vi "translation_control_panel.vi"() -> ()   [LabVIEW 2026]
panel:
  in  "?":bool
  in  "Run":bool
  out "Output":string
  in  "Output File Name":string
  in  "Timeline File":path
  in  "Translation Working Directory":path
  in  "Topology File":path
  in  ".mat File Directory":path
  out "Command Preview":string
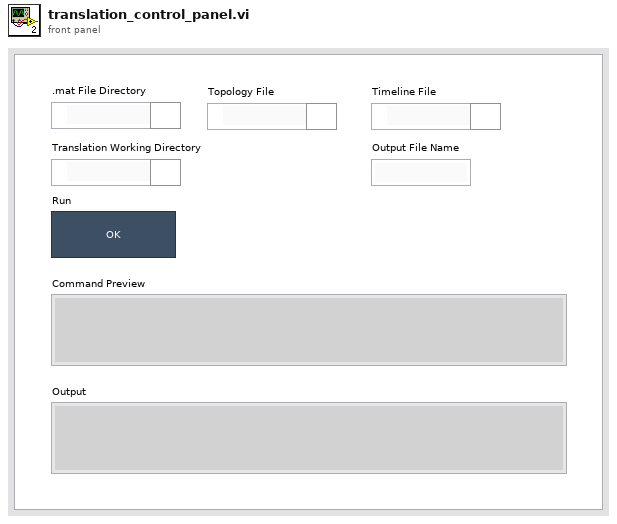
[diagram p1: front panel]
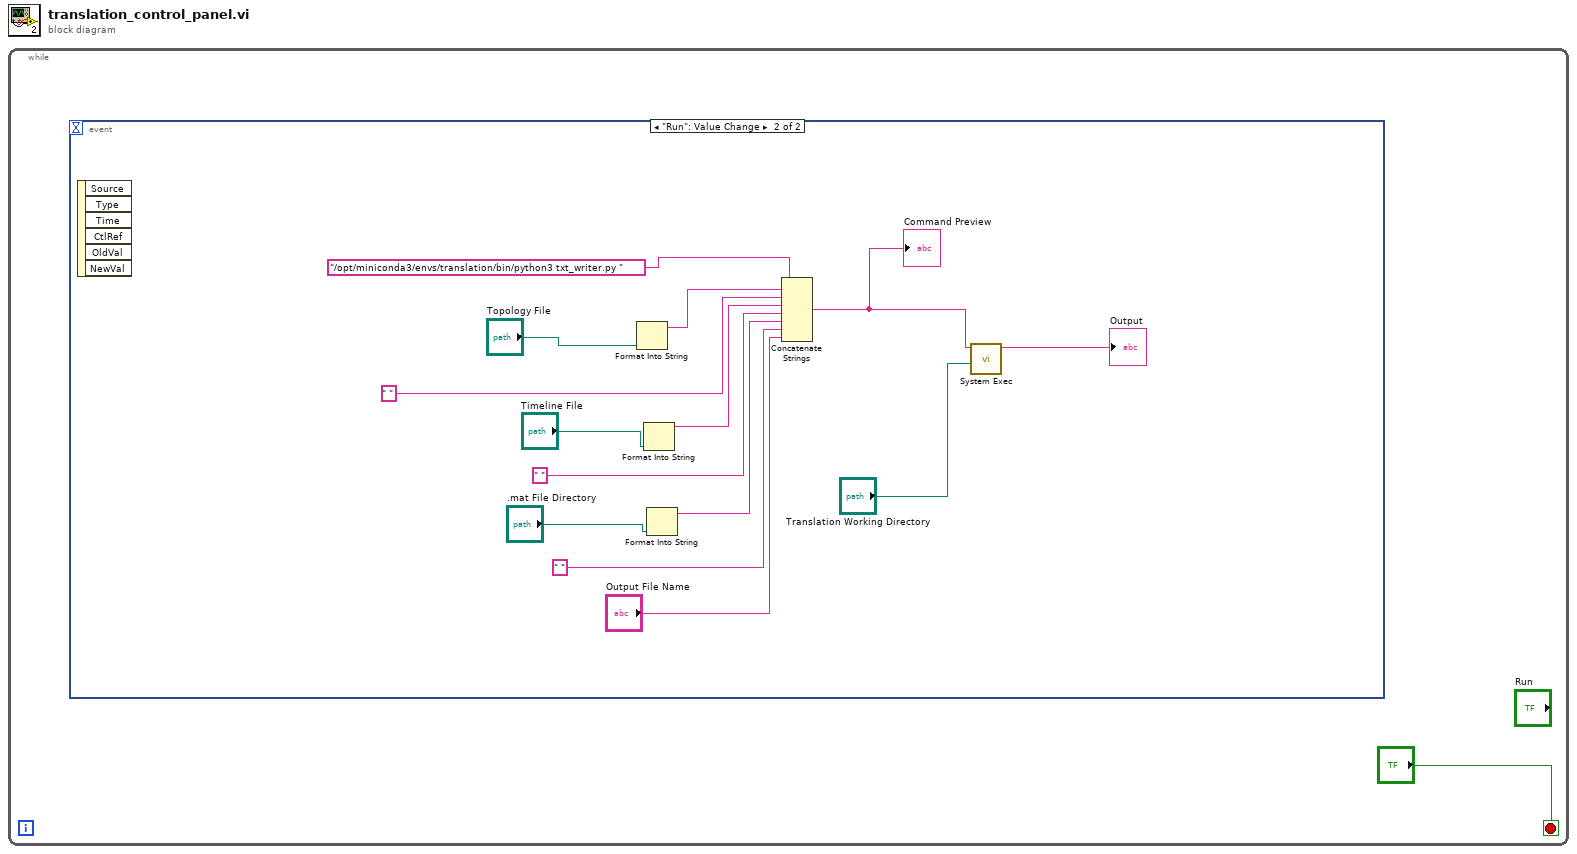
[diagram p0: block diagram]
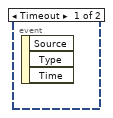
[diagram p2: hidden frame]
diagram:
  n1 = while {
    stop <- "?" stop-if-true
    n2 = event shown="[1] \"Run\": Value Change" {
      selector: _ -> [_ _]
      dyn-events: _ -> [_ _]
      timeout: _ -> [_ _]
      event Timeout {
        n3 = event-data() -> ()  [unwired: 1 in, 3 out]
      }
      event "Run": Value Change {
        n4 = event-data() -> ()  [unwired: 1 in, 6 out]
        n5 = Format Into String("Topology File") -> (resulting string=w7:string)  [unwired: 3 in, 1 out]
        n6 = Format Into String("Timeline File") -> (resulting string=w8:string)  [unwired: 3 in, 1 out]
        n7 = Format Into String(".mat File Directory") -> (resulting string=w13:string)  [unwired: 3 in, 1 out]
        n8 = Concatenate Strings("/opt/miniconda3/envs/translation/bin/python3 txt_writer.py ", w7, " ", w8, " ", w13, " ", "Output File Name") -> (w11:string)
        "Command Preview" <- w11
        n9 = call <vilib>:"System Exec.vi"("working directory"="Translation Working Directory", "command line"=w11) -> ("standard output"=→"Output":string)  [unwired: 6 in, 3 out]
      }
    }
  }
